vi "Create Mapper VIs for Enum.vi"(8 "error in (no error)":errorcluster, 10 "RPC Message Name":string, 11 "Library item in":refnum<vi>) -> (0 "error out":errorcluster, 3 "Library item out":refnum<vi>)   [LabVIEW 2019, in "gRPC Template Creation Utility.lvlib"]
uses:
  gRPC Template Creation Utility.lvlib
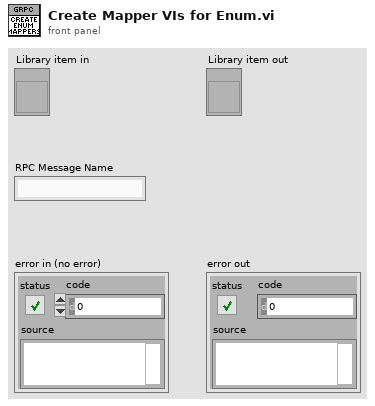
[diagram p1: front panel]
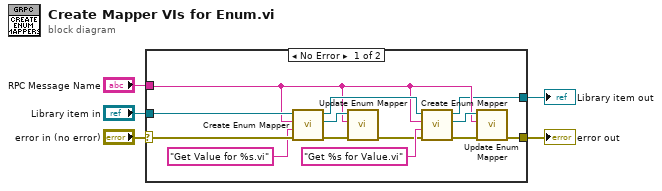
[diagram p0: block diagram]
diagram:
  n1 = case shown="No Error" "error in (no error)" {
    selector: "error in (no error)" -> [w15 w20]
    tunnel: "RPC Message Name" -> [w9 _]
    tunnel: [w6 w20] -> w4
    tunnel: "Library item in" -> [w16 w19]
    tunnel: [w8 w19] -> w1
    frame No Error {
      n2 = call "Create Enum Mapper.vi"("error in"=w15, "format string"="Get Value for %s.vi", "RPC Message Name"=w9, "Library item in"=w16) -> ("error out"=w18:errorcluster, "VI out"=w12:refnum<vi>, "Library item out"=w11:refnum<vi>)  [unwired: 5 in]
      n3 = call "Update Enum Mapper.vi"("error in"=w18, "RPC Message Name"=w9, "VI in"=w12) -> ("error out"=w7:errorcluster)  [unwired: 8 in]
      n4 = call "Create Enum Mapper.vi"("error in"=w7, "format string"="Get %s for Value.vi", "RPC Message Name"=w9, "Library item in"=w11) -> ("error out"=w17:errorcluster, "VI out"=w10:refnum<vi>, "Library item out"=w8:refnum<vi>)  [unwired: 5 in]
      n5 = call "Update Enum Mapper.vi"("error in"=w17, "RPC Message Name"=w9, "VI in"=w10) -> ("error out"=w6:errorcluster)  [unwired: 8 in]
    }
    frame Error {
    }
  }
  "error out" <- w4
  "Library item out" <- w1
